vi "Add Numeric Comparators.vi"(9 "Comparison":string, 10 "Array in":string[](array[string]), 11 "Result Handler":refnum<class "TestStand Result Handler.lvclass">) -> (2 "Array out":string[](array[string]), 3 "Result Handler Out":refnum<class "TestStand Result Handler.lvclass">)   [LabVIEW 2020, in "Astemes_CSVReportPlugin.lvlib" / "TestStand Result Handler.lvclass"]
uses:
  TestStand Result Handler.lvclass
  Columns.ctl
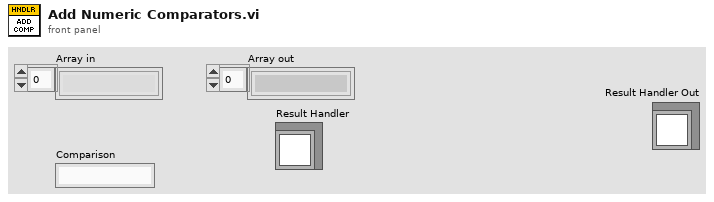
[diagram p1: front panel]
types:
  T1 = typedef "Astemes_CSVReportPlugin.lvlib/TestStand Result Handler.lvclass/Columns.ctl" = enum16{"StepName", "Result", "LowerLimit", "ComparisonTypeLow", "Measurement", "ComparisonTypeHigh", "UpperLimit", "ReportText", "StepType"}
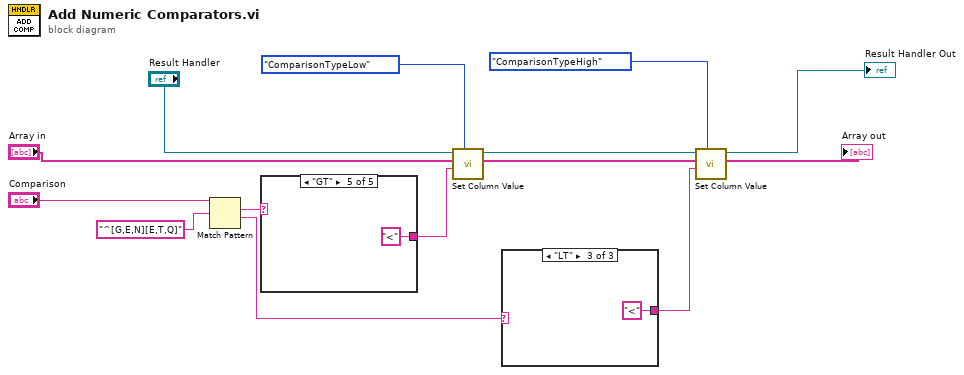
[diagram p0: block diagram]
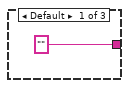
[diagram p2: hidden frame]
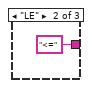
[diagram p3: hidden frame]
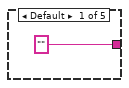
[diagram p4: hidden frame]
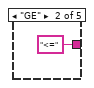
[diagram p5: hidden frame]
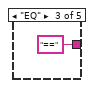
[diagram p6: hidden frame]
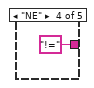
[diagram p7: hidden frame]
diagram:
  n1 = Match Pattern(string="Comparison", regular expression="^[G,E,N][E,T,Q]") -> (match substring=w13:string, after substring=w8:string)  [unwired: 1 in, 2 out]
  n2 = case shown="\"GT\"" w13 {
    tunnel: ["" ("Value") "<=" ("Value") "==" ("Value") "!=" ("Value") "<" ("Value")] -> w12
    frame Default {
    }
    frame "GE" {
    }
    frame "EQ" {
    }
    frame "NE" {
    }
    frame "GT" {
    }
  }
  n3 = call "Set Column Value.vi"("Column"=Columns."ComparisonTypeLow", "Value"=w12, "Row In"="Array in", "Result Handler"="Result Handler") -> ("Row Out"=w2:string[], "Result Handler Out"=w10:refnum<class "TestStand Result Handler.lvclass">)  [unwired: 6 in]
  n4 = case shown="\"LT\"" w8 {
    tunnel: ["" ("Value") "<=" ("Value") "<" ("Value")] -> w9
    frame Default {
    }
    frame "LE" {
    }
    frame "LT" {
    }
  }
  n5 = call "Set Column Value.vi"("Column"=Columns."ComparisonTypeHigh", "Value"=w9, "Row In"=w2, "Result Handler"=w10) -> ("Row Out"=→"Array out":string[], "Result Handler Out"=→"Result Handler Out":refnum<class "TestStand Result Handler.lvclass">)  [unwired: 6 in]
